vi "Main - Manages 3rd Party Slaves.vi"(8 "error in (no error)":errorcluster, 11 "Node Ptr":u64 format="%.0x") -> (0 "error out":errorcluster)   [LabVIEW 2020, in "SEECD System Explorer.lvlib"]
uses:
  SEECD System Explorer.lvlib
  <vilib>/NI VeriStand/Custom Device API/Custom Device Target Type.ctl
  Applications/Utilities/ECAT Files.ctl
  <vilib>/NI VeriStand/Custom Device API/Custom Device API.lvlib
panel:
  in  "--> Upload Profile to Target-->":bool
  in  "Found device profiles on RT-Target":i32(listbox)=-1
  in  "Found device profiles on Host":i32(listbox)=-1
  in  "Update List":bool
  in  "Tag":string
  in  "Close":bool
  in  "Help":bool
  in  "Import":bool
  in  "Import to RT target":bool=TRUE caption="Import to the real-time target"
  in  "Import to host PC":bool=TRUE caption="Import to the host computer"
  in  "Found device profiles":i32(listbox)=6
  in  "Select a device profile or file path":path
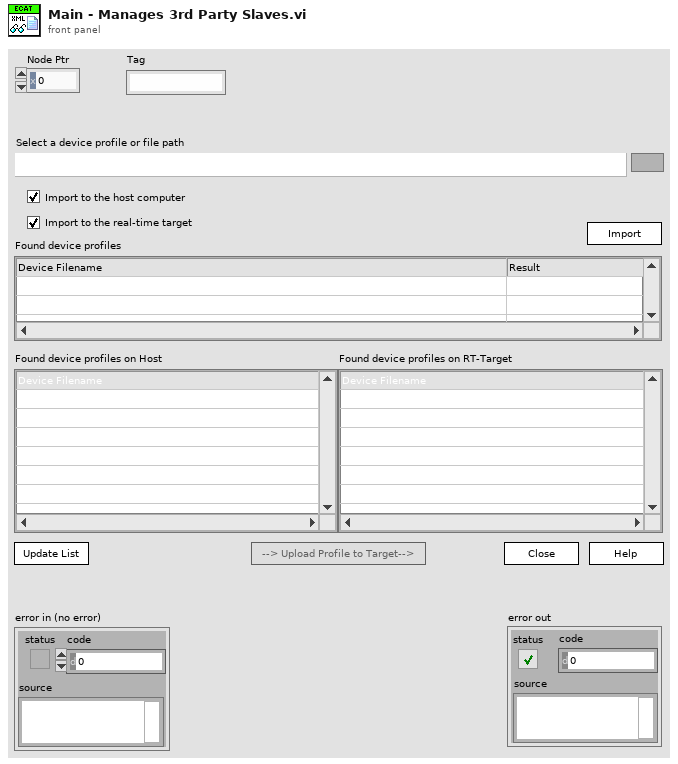
[diagram p1: front panel]
types:
  T1 = typedef "Custom Device API.lvlib/Custom Device Target Type.ctl" = enum16{"PharLap", "VxWorks", "Windows", "Linux_32_ARM", "Linux_x64"}
  T2 = enum8{"Enabled", "Disabled", "Disabled and Grayed Out"}
  T3 = typedef "SEECD System Explorer.lvlib/ECAT Files.ctl" = enum16{"niECATLVProvider.mxx", "indcomecat.chm", "Providers DD", "Shared DD"}
  T4 = typedef "Custom Device API.lvlib/Custom Device Item Ref.ctl" = u64
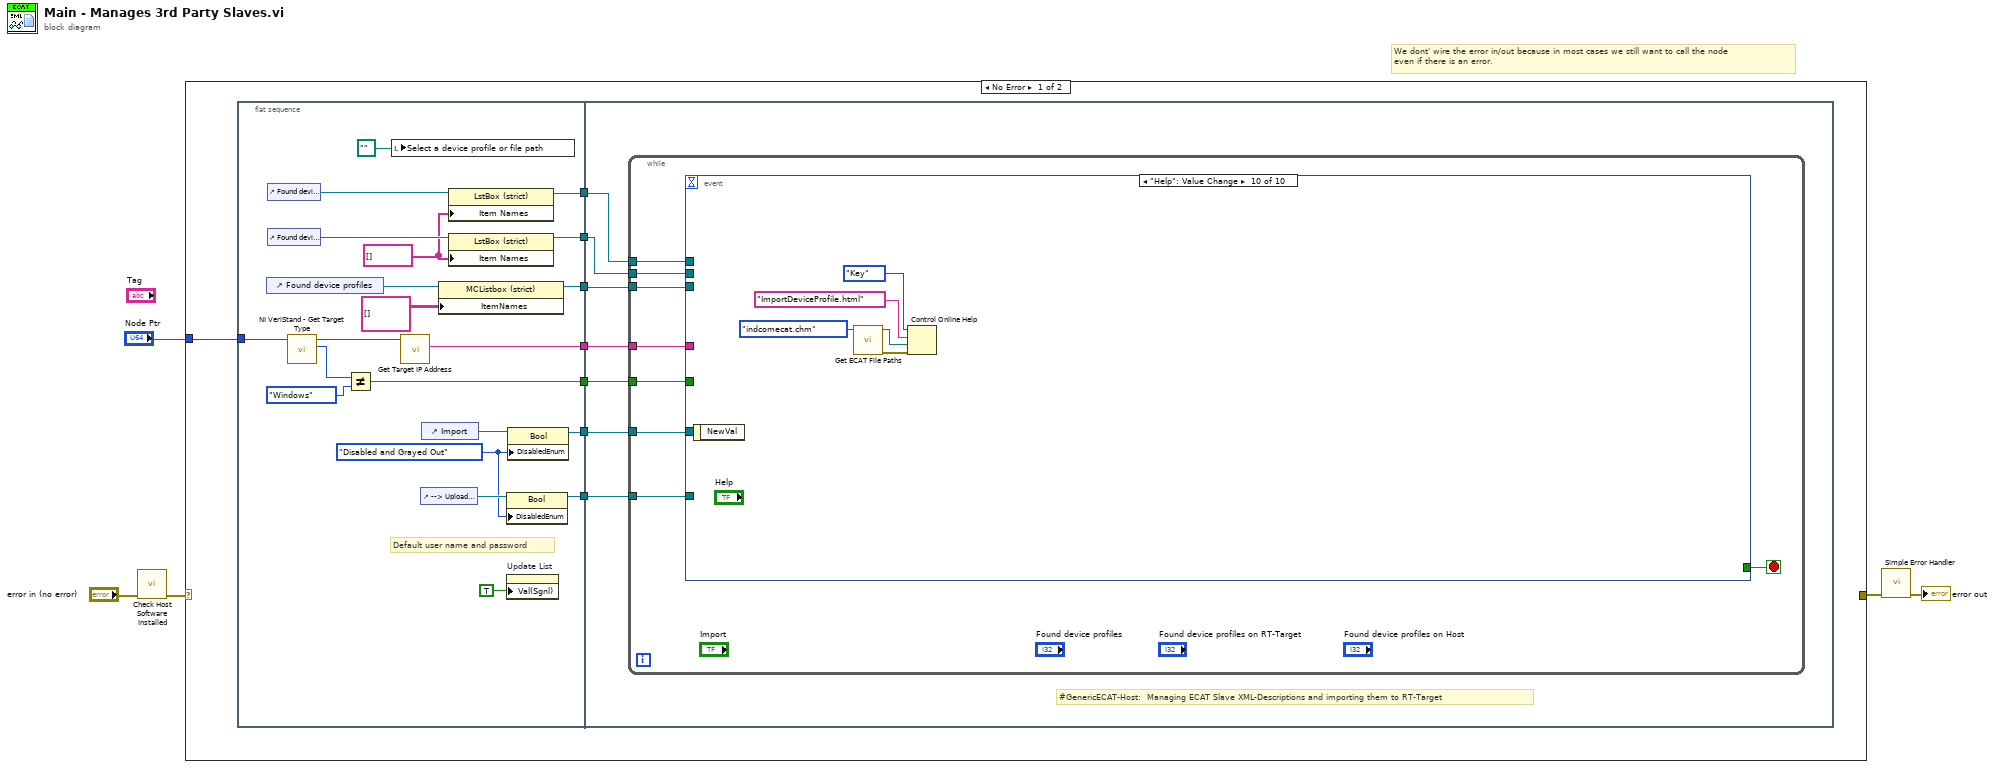
[diagram p0: block diagram]
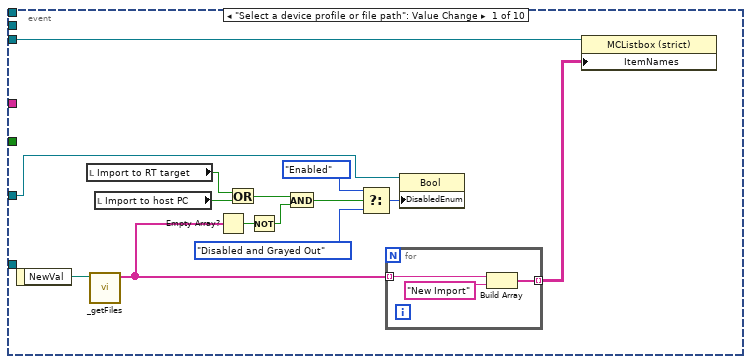
[diagram p2: hidden frame]
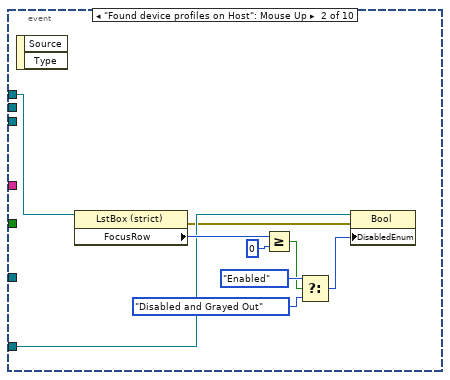
[diagram p3: hidden frame]
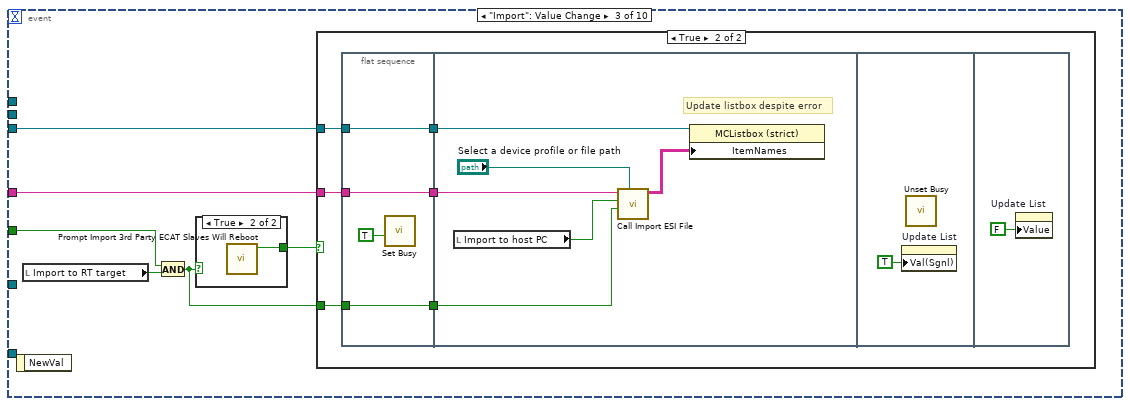
[diagram p4: hidden frame]
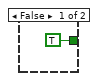
[diagram p6: hidden frame]
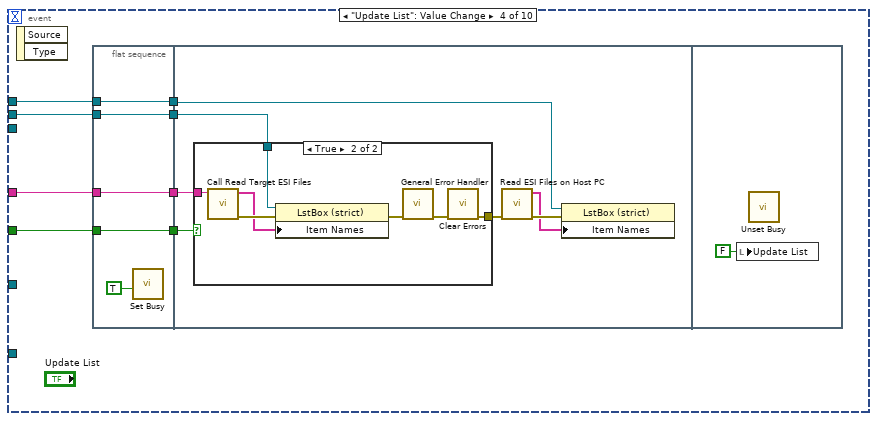
[diagram p7: hidden frame]
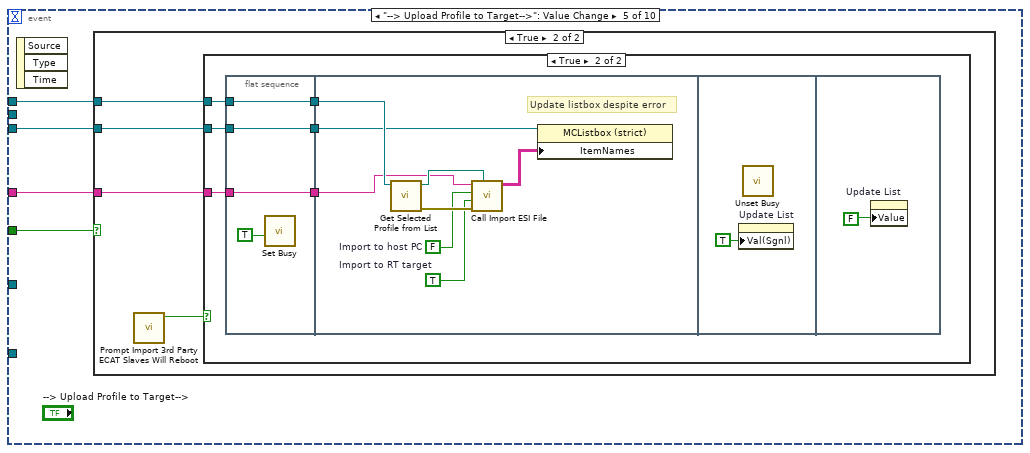
[diagram p9: hidden frame]
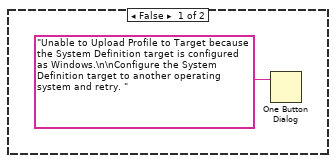
[diagram p10: hidden frame]
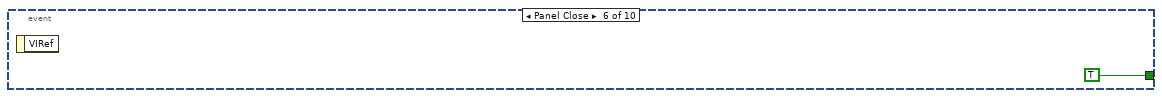
[diagram p12: hidden frame]
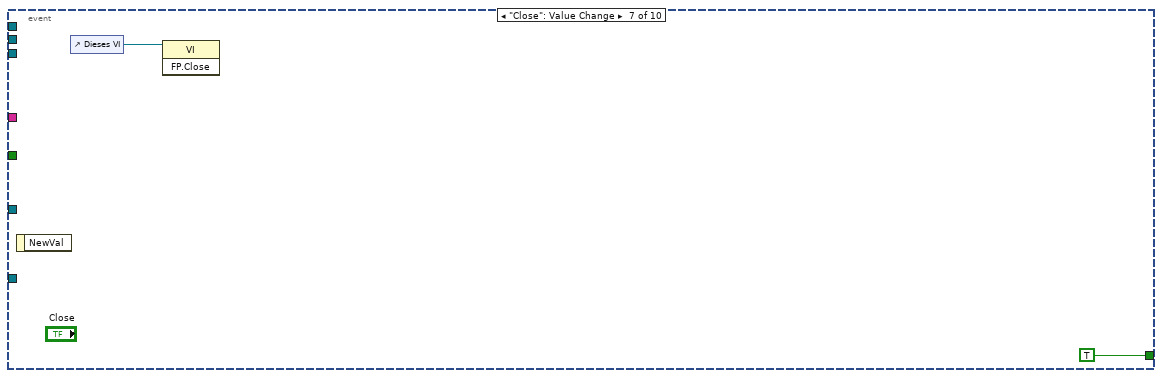
[diagram p13: hidden frame]
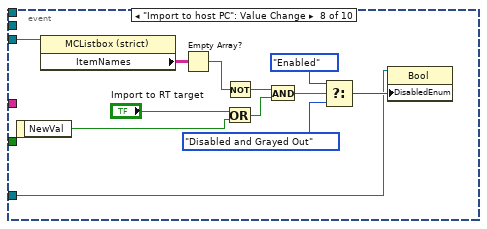
[diagram p14: hidden frame]
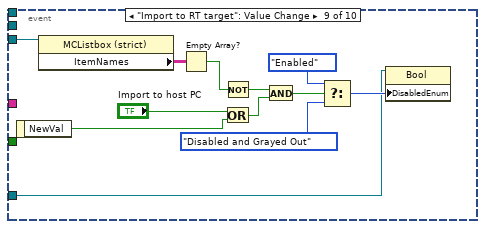
[diagram p15: hidden frame]
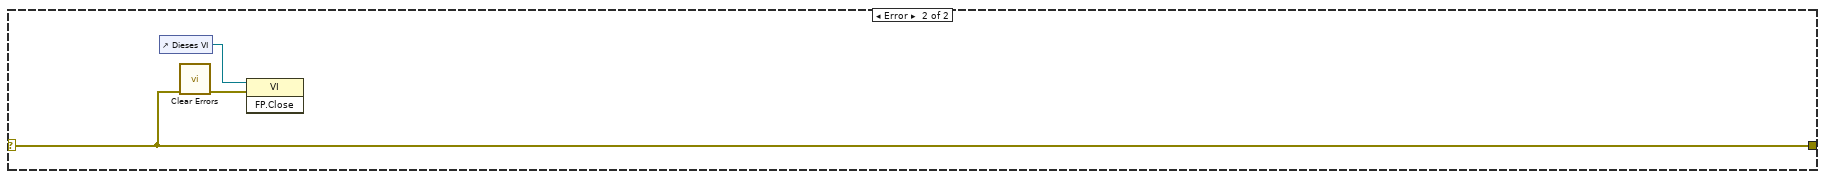
[diagram p16: hidden frame]
diagram:
  # "We dont' wire the error in/out because in most cases we still want to call the node\neven if there is an error."
  n1 = call "Check Host Software Installed.vi"("error in"="error in (no error)") -> ("error out"=w1:errorcluster)  [unwired: 10 in]
  n2 = case shown="No Error" w1 {
    selector: w1 -> [_ w191]
    tunnel: [_ w191] -> w4
    tunnel: "Node Ptr" -> [w13 _]
    frame No Error {
      n3 = flat-sequence {
        tunnel: [w30] -> w12
        tunnel: [w32] -> w11
        tunnel: w13 -> [w18]
        tunnel: [w26] -> w10
        tunnel: [w25] -> w9
        tunnel: [w21] -> w8
        tunnel: [w15] -> w7
        tunnel: [w14] -> w6
        tunnel: w12 -> [w41]
        tunnel: w11 -> [w40]
        tunnel: w10 -> [w39]
        tunnel: w9 -> [w38]
        tunnel: w8 -> [w37]
        tunnel: w7 -> [w36]
        tunnel: w6 -> [w35]
        frame #0 {
          w24 = string[] []
          w22 = T2."Disabled and Grayed Out" ("Disabled")
          # "Default user name and password"
          n4 = control-ref of="Found device profiles"() -> (w33:refnum<vi>)
          n5 = control-ref of="Found device profiles on Host"() -> (w29:refnum<vi>)
          n6 = control-ref of="Found device profiles on RT-Target"() -> (w28:refnum<vi>)
          n7 = call <vilib>:"NI VeriStand - Get Target Type.vi"("Item Ref in"=w18) -> ("Target Type"=w16:T1, "Item Ref out"=w17:T4)  [unwired: 8 in, 1 out]
          n8 = Not Equal?(x=w16, y=Custom_Device_Target_Type."Windows") -> (x != y?=w14:bool)
          n9 = local write "Select a device profile or file path"(path "" ("Device Profile Filename or Path")) -> ()
          n10 = call "Get Target IP Address.vi"("Item Ref in"=w17) -> ("Target IP Address"=w15:string)  [unwired: 8 in, 2 out]
          n11 = control-ref of="--> Upload Profile to Target-->"() -> (w23:refnum<vi>)
          n12 = control-ref of="Import"() -> (w31:refnum<vi>)
          n13 = property on="Property Node" class="MCListbox (strict)"(reference=w33, "ItemNames"=string[][] [] ("Item Names")) -> (reference out=w32:refnum<vi>)  [unwired: 1 in, 1 out]
          n14 = property on="Property Node" class="LstBox (strict)"(reference=w29, "Item Names"=w24) -> (reference out=w25:refnum<vi>)  [unwired: 1 in, 1 out]
          n15 = property on="Property Node" class="LstBox (strict)"(reference=w28, "Item Names"=w24) -> (reference out=w26:refnum<vi>)  [unwired: 1 in, 1 out]
          n16 = property on="Property Node" class="Bool"(reference=w23, "DisabledEnum"=w22) -> (reference out=w21:refnum<vi>)  [unwired: 1 in, 1 out]
          n17 = property on="Update List" class="Bool (strict)"("Val(Sgnl)"=TRUE ("Wert (signalisierend)")) -> ()  [unwired: 2 in, 2 out]
          n18 = property on="Property Node" class="Bool"(reference=w31, "DisabledEnum"=w22) -> (reference out=w30:refnum<vi>)  [unwired: 1 in, 1 out]
        }
        frame #1 {
          # "#GenericECAT-Host:  Managing ECAT Slave XML-Descriptions and importing them to RT-Target"
          n19 = while {
            tunnel: w41 -> [w49]
            tunnel: w40 -> [w48]
            tunnel: w39 -> [w46]
            tunnel: w38 -> [w45]
            tunnel: w37 -> [w44]
            tunnel: w36 -> [w43]
            tunnel: w35 -> [w42]
            stop <- w47 stop-if-true
            n20 = event shown="[9] \"Help\": Value Change" {
              selector: _ -> [_ _ _ _ _ _ _ _ _ _]
              dyn-events: _ -> [_ _ _ _ _ _ _ _ _ _]
              timeout: _ -> [_ _ _ _ _ _ _ _ _ _]
              tunnel: [_ _ _ _ _ TRUE TRUE _ _ _] -> w47
              tunnel: w49 -> [w50 _ _ _ _ _ _ w170 w182 _]
              tunnel: w48 -> [w52 _ w81 _ w133 _ _ w165 w178 _]
              tunnel: w46 -> [_ _ _ w108 _ _ _ _ _ _]
              tunnel: w45 -> [_ w75 _ w106 w132 _ _ _ _ _]
              tunnel: w44 -> [_ w69 _ _ _ _ _ _ _ _]
              tunnel: w43 -> [_ _ w76 w105 w131 _ _ _ _ _]
              tunnel: w42 -> [_ _ w77 w102 w130 _ _ _ _ _]
              event "Select a device profile or file path": Value Change {
                n21 = event-data() -> ("NewVal"=w60:path)  [unwired: 1 out]
                n22 = local read "Import to RT target"() -> (w59:bool)
                n23 = call "_getFiles.vi"("Selected path"=w60) -> ("Import files"=w53:string[])  [unwired: 6 in]
                n24 = local read "Import to host PC"() -> (w58:bool)
                n25 = Empty Array?(array=w53) -> (empty?=w54:bool)
                n26 = Or(x=w59, y=w58) -> (x .or. y?=w57:bool)
                n27 = Not(x=w54) -> (.not. x?=w56:bool)
                n28 = And(x=w57, y=w56) -> (x .and. y?=w55:bool)
                n29 = Select(t=T2."Enabled" ("Disabled"), s=w55, f=T2."Disabled and Grayed Out" ("Disabled")) -> (s? t:f=w61:T2)
                n30 = for {
                  tunnel: w53 -> [w64] mode=indexing
                  tunnel: [w65] -> w51 mode=indexing
                  n31 = Build Array(w64, "New Import" ("element")) -> (w65:string[])
                }
                n32 = property on="Property Node" class="Bool"(reference=w50, "DisabledEnum"=w61) -> ()  [unwired: 1 in, 2 out]
                n33 = property on="Property Node" class="MCListbox (strict)"(reference=w52, "ItemNames"=w51) -> ()  [unwired: 1 in, 2 out]
              }
              event "Found device profiles on Host": Mouse Up {
                n34 = event-data() -> ()  [unwired: 3 out]
                n35 = property on="Property Node" class="LstBox (strict)"(reference=w75) -> (error out=w67:errorcluster, "FocusRow"=w74:i32)  [unwired: 1 in, 1 out]
                n36 = Greater Or Equal?(x=w74, y=0) -> (x >= y?=w68:bool)
                n37 = Select(t=T2."Enabled" ("Disabled"), s=w68, f=T2."Disabled and Grayed Out" ("Disabled")) -> (s? t:f=w70:T2)
                n38 = property on="Property Node" class="Bool"(reference=w69, error in=w67, "DisabledEnum"=w70) -> ()  [unwired: 2 out]
              }
              event "Import": Value Change {
                n39 = event-data() -> ()  [unwired: 2 out]
                n40 = local read "Import to RT target"() -> (w79:bool)
                n41 = And(x=w77, y=w79) -> (x .and. y?=w78:bool)
                n42 = case shown="True" w78 {
                  tunnel: [TRUE ("Continue?") w101] -> w80
                  frame False {
                  }
                  frame True {
                    n43 = call "Prompt Import 3rd Party ECAT Slaves Will Reboot.vi"() -> ("Continue?"=w101:bool)  [unwired: 11 in]
                  }
                }
                n44 = case shown="True" w80 {
                  tunnel: w81 -> [_ w86]
                  tunnel: w78 -> [_ w85]
                  tunnel: w76 -> [_ w82]
                  frame False {
                  }
                  frame True {
                    n45 = flat-sequence {
                      tunnel: [w91] -> w87
                      tunnel: w86 -> [w91]
                      tunnel: w85 -> [w89]
                      tunnel: [w89] -> w84
                      tunnel: [w88] -> w83
                      tunnel: w82 -> [w88]
                      tunnel: w87 -> [w97]
                      tunnel: w84 -> [w93]
                      tunnel: w83 -> [w92]
                      frame #0 {
                        n46 = call <vilib>:"Set Busy.vi"("disable click? (T)"=TRUE) -> ()  [unwired: 3 in, 8 out]
                      }
                      frame #1 {
                        # "Update listbox despite error"
                        n47 = local read "Import to host PC"() -> (w94:bool)
                        n48 = call "Call Import ESI File.vi"("Select a device profile or file path"="Select a device profile or file path", "Import to RT target"=w93, "Import to host PC"=w94, "Target IP Address"=w92) -> ("result out"=w96:string[][])  [unwired: 6 in, 1 out]
                        n49 = property on="Property Node" class="MCListbox (strict)"(reference=w97, "ItemNames"=w96) -> ()  [unwired: 1 in, 2 out]
                      }
                      frame #2 {
                        n50 = property on="Update List" class="Bool (strict)"("Val(Sgnl)"=TRUE ("Wert (signalisierend)")) -> ()  [unwired: 2 in, 2 out]
                        n51 = call <vilib>:"Unset Busy.vi"() -> ()  [unwired: 2 in, 10 out]
                      }
                      frame #3 {
                        n52 = property on="Update List" class="Bool (strict)"("Value"=FALSE ("Wert (signalisierend)")) -> ()  [unwired: 2 in, 2 out]
                      }
                    }
                  }
                }
              }
              event "Update List": Value Change {
                n53 = event-data() -> ()  [unwired: 3 out]
                n54 = flat-sequence {
                  tunnel: [w113] -> w109
                  tunnel: w108 -> [w113]
                  tunnel: [w112] -> w107
                  tunnel: w106 -> [w112]
                  tunnel: w105 -> [w111]
                  tunnel: [w111] -> w104
                  tunnel: [w110] -> w103
                  tunnel: w102 -> [w110]
                  tunnel: w109 -> [w120]
                  tunnel: w107 -> [w121]
                  tunnel: w104 -> [w116]
                  tunnel: w103 -> [w115]
                  frame #0 {
                    n55 = call <vilib>:"Set Busy.vi"("disable click? (T)"=TRUE) -> ()  [unwired: 3 in, 8 out]
                  }
                  frame #1 {
                    n56 = case shown="True" w115 {
                      tunnel: w120 -> [_ w128]
                      tunnel: [_ w127] -> w117
                      tunnel: w116 -> [_ w126]
                      frame False {
                      }
                      frame True {
                        n57 = call "Call Read Target ESI Files.vi"("IP address"=w126) -> ("error out"=w125:errorcluster, "Existing Target Profiles"=w124:string[])  [unwired: 9 in]
                        n58 = property on="Property Node" class="LstBox (strict)"(reference=w128, error in=w125, "Item Names"=w124) -> (error out=w123:errorcluster)  [unwired: 1 out]
                        n59 = call <vilib>:"General Error Handler.vi"("error in (no error)"=w123) -> ("error out"=w122:errorcluster)  [unwired: 10 in, 4 out]
                        n60 = call <vilib>:"Clear Errors.vi"("error in (no error)"=w122) -> ("error out"=w127:errorcluster)  [unwired: 5 in, 1 out]
                      }
                    }
                    n61 = call "Read ESI Files on Host PC.vi"("error in (no error)"=w117) -> ("error out"=w119:errorcluster, "Existing Host Profiles"=w118:string[])  [unwired: 9 in]
                    n62 = property on="Property Node" class="LstBox (strict)"(reference=w121, error in=w119, "Item Names"=w118) -> ()  [unwired: 2 out]
                  }
                  frame #2 {
                    n63 = local write "Update List"(FALSE) -> ()
                    n64 = call <vilib>:"Unset Busy.vi"() -> ()  [unwired: 2 in, 10 out]
                  }
                }
              }
              event "--> Upload Profile to Target-->": Value Change {
                n65 = event-data() -> ()  [unwired: 4 out]
                n66 = case shown="True" w130 {
                  tunnel: w133 -> [_ w138]
                  tunnel: w132 -> [_ w137]
                  tunnel: w131 -> [_ w135]
                  frame False {
                    n67 = One Button Dialog(message="Unable to Upload Profile to Target because the System Definition target is configured as Windows.\n\nConfigure the System Definition target to another operating system and retry. ") -> ()  [unwired: 1 in, 1 out]
                  }
                  frame True {
                    n68 = call "Prompt Import 3rd Party ECAT Slaves Will Reboot.vi"() -> ("Continue?"=w136:bool)  [unwired: 11 in]
                    n69 = case shown="True" w136 {
                      tunnel: w138 -> [_ w142]
                      tunnel: w137 -> [_ w141]
                      tunnel: w135 -> [_ w140]
                      frame False {
                      }
                      frame True {
                        n70 = flat-sequence {
                          tunnel: [w148] -> w144
                          tunnel: w142 -> [w148]
                          tunnel: [w146] -> w143
                          tunnel: w141 -> [w146]
                          tunnel: w140 -> [w145]
                          tunnel: [w145] -> w139
                          tunnel: w144 -> [w150]
                          tunnel: w143 -> [w155]
                          tunnel: w139 -> [w149]
                          frame #0 {
                            n71 = call <vilib>:"Set Busy.vi"("disable click? (T)"=TRUE) -> ()  [unwired: 3 in, 8 out]
                          }
                          frame #1 {
                            w152 = TRUE  # Import to RT target
                            w153 = FALSE  # Import to host PC
                            # "Update listbox despite error"
                            n72 = call "Get Selected Profile from List.vi"("Referenz"=w155) -> ("error out"=w156:errorcluster, "Selected Profile Path"=w154:path)  [unwired: 9 in]
                            n73 = call "Call Import ESI File.vi"("Select a device profile or file path"=w154, "error in"=w156, "Import to RT target"=w152, "Import to host PC"=w153, "Target IP Address"=w149) -> ("result out"=w151:string[][])  [unwired: 5 in, 1 out]
                            n74 = property on="Property Node" class="MCListbox (strict)"(reference=w150, "ItemNames"=w151) -> ()  [unwired: 1 in, 2 out]
                          }
                          frame #2 {
                            n75 = property on="Update List" class="Bool (strict)"("Val(Sgnl)"=TRUE ("Wert (signalisierend)")) -> ()  [unwired: 2 in, 2 out]
                            n76 = call <vilib>:"Unset Busy.vi"() -> ()  [unwired: 2 in, 10 out]
                          }
                          frame #3 {
                            n77 = property on="Update List" class="Bool (strict)"("Value"=FALSE ("Wert (signalisierend)")) -> ()  [unwired: 2 in, 2 out]
                          }
                        }
                      }
                    }
                  }
                }
              }
              event Panel Close {
                n78 = event-data() -> ()  [unwired: 2 out]
              }
              event "Close": Value Change {
                n79 = event-data() -> ()  [unwired: 2 out]
                n80 = control-ref of="Dieses VI"() -> (w160:refnum<vi>)
                n81 = invoke class="VI" method="FP.Close"(reference=w160) -> ()  [unwired: 2 in, 3 out]
              }
              event "Import to host PC": Value Change {
                n82 = event-data() -> ("NewVal"=w167:bool)  [unwired: 1 out]
                n83 = property on="Property Node" class="MCListbox (strict)"(reference=w165) -> ("ItemNames"=w164:string[][])  [unwired: 1 in, 2 out]
                n84 = Empty Array?(array=w164) -> (empty?=w163:bool)
                n85 = Not(x=w163) -> (.not. x?=w166:bool)
                n86 = Or(x="Import to RT target", y=w167) -> (x .or. y?=w162:bool)
                n87 = And(x=w166, y=w162) -> (x .and. y?=w168:bool)
                n88 = Select(t=T2."Enabled" ("Disabled"), s=w168, f=T2."Disabled and Grayed Out" ("Disabled")) -> (s? t:f=w171:T2)
                n89 = property on="Property Node" class="Bool"(reference=w170, "DisabledEnum"=w171) -> ()  [unwired: 1 in, 2 out]
              }
              event "Import to RT target": Value Change {
                n90 = event-data() -> ("NewVal"=w181:bool)  [unwired: 1 out]
                n91 = property on="Property Node" class="MCListbox (strict)"(reference=w178) -> ("ItemNames"=w177:string[][])  [unwired: 1 in, 2 out]
                n92 = Empty Array?(array=w177) -> (empty?=w176:bool)
                n93 = Not(x=w176) -> (.not. x?=w175:bool)
                n94 = Or(x="Import to host PC", y=w181) -> (x .or. y?=w174:bool)
                n95 = And(x=w175, y=w174) -> (x .and. y?=w179:bool)
                n96 = Select(t=T2."Enabled" ("Disabled"), s=w179, f=T2."Disabled and Grayed Out" ("Disabled")) -> (s? t:f=w183:T2)
                n97 = property on="Property Node" class="Bool"(reference=w182, "DisabledEnum"=w183) -> ()  [unwired: 1 in, 2 out]
              }
              event "Help": Value Change {
                n98 = event-data() -> ()  [unwired: 2 out]
                n99 = call "Get ECAT File Paths.vi"("ECAT File"=ECAT_Files."indcomecat.chm") -> ("error out"=w188:errorcluster, "File Path"=w187:path)  [unwired: 9 in]
                n100 = Control Online Help(1:w188, 2:w187, 3:"ImportDeviceProfile.html" ("String to search for"), 4:enum16{"Contents", "Key", "Close"}."Key" ("Operation")) -> ()  [unwired: 1 out]
              }
            }
          }
        }
      }
    }
    frame Error {
      n101 = control-ref of="Dieses VI"() -> (w193:refnum<vi>)
      n102 = call <vilib>:"Clear Errors.vi"("error in (no error)"=w191) -> ("error out"=w192:errorcluster)  [unwired: 5 in, 1 out]
      n103 = invoke class="VI" method="FP.Close"(reference=w193, error in=w192) -> ()  [unwired: 1 in, 3 out]
    }
  }
  n104 = call <vilib>:"Simple Error Handler.vi"("error in (no error)"=w4) -> ("error out"=→"error out":errorcluster)  [unwired: 4 in, 4 out]
